vi "FuncVI-SineWave.vi"(5 "InstanceRef":T2, 9 "arg list":T1[](array[typedef]) {"num" format="%.2f"}) -> (0 "error out":bool, 3 "result":T1 {"num" format="%.2f"})   [LabVIEW 2021]
doc: "::: CalcExpress Toolkit :::\nCopyright (c) 2000-2026 Konstantin Shifershteyn. All rights reserved."
uses:
  cetypes.llb/CalcExpress Function Argument Info.ctl
  cetypes.llb/CalcExpress Instance RefNum.ctl
  <vilib>/Analysis/NI_AALBase.lvlib
panel:
  in  "max arg num":i32=5
  in  "min arg num":i32=1
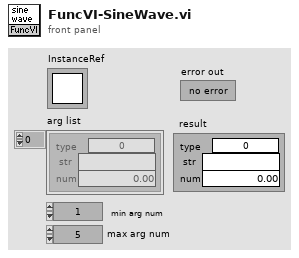
[diagram p1: front panel]
types:
  T1 = typedef "CalcExpress Function Argument Info.ctl" = cluster{"type":u32, "str":string, "num":dbl}
  T2 = typedef "CalcExpress Instance RefNum.ctl" = refnum<k1>
  T3 = enum8{"String", "DBL Number", "identifier", "1D Array of DBL", "2D Array of DBL", "CDB Number", "1D Array of CDB", "2D Array of CDB", "1D Array of String", "2D Array of String", "Unknown data type"}
  T4 = cluster{"index":i32, "type":enum8{"String", "DBL Number", "identifier", "1D Array of DBL", "2D Array of DBL", "CDB Number", "1D Array of CDB", "2D Array of CDB", "Unknown data type"}, "default num":dbl, "default str":string}[]
  T5 = cluster{"num list[0]":dbl, "num list[1]":dbl, "num list[2]":dbl, "num list[3]":dbl, "num list[4]":dbl}
  T6 = typedef "VarMan Variable Context Handle.ctl" = i32
  T7 = cluster{"type":enum8{"String", "DBL Number", "identifier", "1D Array of DBL", "2D Array of DBL", "CDB Number", "1D Array of CDB", "2D Array of CDB", "1D Array of String", "2D Array of String", "Unknown data type"}, string, "phase out":dbl}
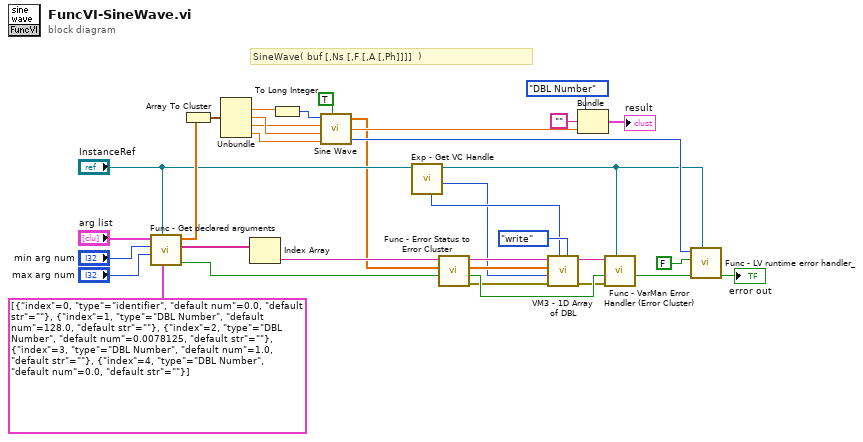
[diagram p0: block diagram]
diagram:
  # "SineWave( buf [,Ns [,F [,A [,Ph]]]]  )"
  n1 = call "Func - Get declared arguments.vi"("arg descriptors"=T4 [{"index"=0, "type"=enum."identifier", "default num"=0.0, "default str"=""}, {"index"=1, "type"=enum."DBL Number", "default num"=128.0, "default str"=""}, {"index"=2, "type"=enum."DBL Number", "default num"=0.0078125, "default str"=""}, {"index"=3, "type"=enum."DBL Number", "default num"=1.0, "default str"=""}, {"index"=4, "type"=enum."DBL Number", "default num"=0.0, "default str"=""}] ("args descriptors"), "InstanceRef"="InstanceRef", "max arg num"="max arg num", "min arg num"="min arg num", "arg list"="arg list") -> ("error out"=w2:bool, "str list"=w24:string[], "num list"=w30:dbl[])  [unwired: 3 in, 1 out]
  n2 = Array To Cluster(array=w30) -> (cluster=w29:T5)
  n3 = Unbundle(w29) -> ("num list[1]"=w22:dbl, "num list[2]"=w21:dbl, "num list[3]"=w20:dbl, "num list[4]"=w19:dbl)  [unwired: 1 out]
  n4 = Index Array(array=w24) -> (element=w5:string)  [unwired: 1 in]
  n5 = To Long Integer(number=w22) -> (32bit integer=w28:i32)
  n6 = call <vilib>:"Sine Wave.vi"("samples"=w28, "amplitude"=w20, "frequency"=w21, "phase in"=w19, "reset phase"=TRUE) -> ("sine wave"=w4:dbl[], "phase out"=w27:dbl, "error"=w18:i32)
  n7 = call "Exp - Get VC Handle.vi"("InstanceRef"="InstanceRef") -> ("writer ID"=w3:u32, "dup InstanceRef"=w7:T2, "VC Handle"=w6:T6)  [unwired: 5 in, 1 out]
  n8 = call "Func - Error Status to Error Cluster.vi"("error status in"=w2) -> ("Error Cluster out"=w11:errorcluster, "error status out"=w12:bool)  [unwired: 9 in]
  n9 = call "VM3 - 1D Array of DBL.vi"("cmd (read)"=enum16{"create", "destroy", "write", "read"}."write", "VC Handle"=w6, "error in"=w11, "writer ID"=w3, "value in"=w4, "name_spec"=w5) -> ("error out"=w8:errorcluster, "dup name_spec"=w9:string)  [unwired: 2 in, 2 out]
  n10 = Bundle("type"=T3."DBL Number", "", "phase out"=w27) -> (→"result":T7)  [unwired: 1 in]
  n11 = call "Func - VarMan Error Handler (Error Cluster).vi"("InstanceRef"=w7, "VarMan VI error in"=w8, "error status before"=w12, "var name"=w9) -> ("FuncVI error out"=w1:bool)  [unwired: 5 in, 2 out]
  n12 = call "Func - LV runtime error handler_.vi"("InstanceRef"=w7, "error in"=w1, "Gen CE error?"=FALSE, "LabVIEW error code"=w18) -> ("error out"=→"error out":bool)  [unwired: 7 in]
